vi "Exp - exec function error message.vi"(6 "error in":errorcluster, 9 "func name":string) -> (0 "error out":errorcluster, 1 "error message":string)   [LabVIEW 2021]
doc: "::: CalcExpress Toolkit :::\nCopyright (c) 2000-2026 Konstantin Shifershteyn. All rights reserved."
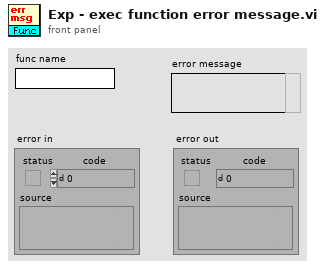
[diagram p1: front panel]
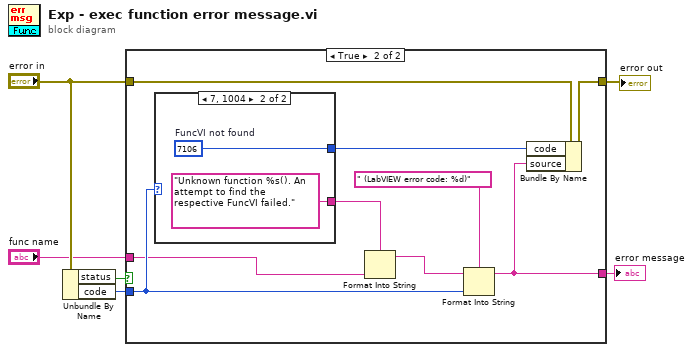
[diagram p0: block diagram]
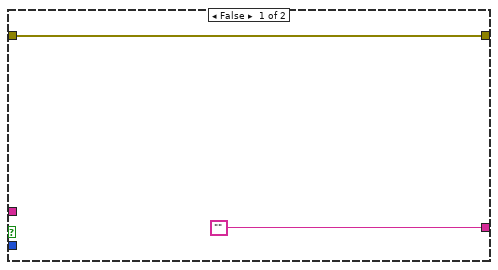
[diagram p2: hidden frame]
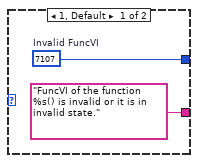
[diagram p3: hidden frame]
diagram:
  n1 = Unbundle By Name("error in") -> ("status"=w6:bool, "code"=w5:i32)
  n2 = case shown="True" w6 {
    tunnel: w5 -> [_ w16]
    tunnel: [w8 w13] -> w3
    tunnel: "error in" -> [w8 w12]
    tunnel: ["" ("Empty String Constant") w11] -> w2
    tunnel: "func name" -> [_ w9]
    frame False {
    }
    frame True {
      n3 = case shown="7, 1004" w16 {
        tunnel: ["FuncVI of the function %s() is invalid or it is in invalid state." "Unknown function %s(). An attempt to find the respective FuncVI failed."] -> w15
        tunnel: [w18 w20] -> w10
        frame 1, Default {
          w18 = 7107  # Invalid FuncVI
        }
        frame 7, 1004 {
          w20 = 7106  # FuncVI not found
        }
      }
      n4 = Format Into String(format string=w15, w9) -> (resulting string=w14:string)  [unwired: 2 in, 1 out]
      n5 = Format Into String(format string=" (LabVIEW error code: %d)", initial string=w14, w16) -> (resulting string=w11:string)  [unwired: 1 in, 1 out]
      n6 = Bundle By Name(cluster=w12, "code"=w10, "source"=w11) -> (w13:errorcluster)
    }
  }
  "error out" <- w3
  "error message" <- w2
